vi "Check Registry.vi"(10 "registry":T1[](array[typedef]), 11 "indicator data in":refnum<data-value>) -> (2 "empty registry?":bool, 3 "indicator data out":refnum<data-value>)   [LabVIEW 2018, in "GLog.lvlib" / "UI Updater.lvlib"]
uses:
  UI Updater.lvlib
  Handler Registration.ctl
  Indicator Data.ctl
panel:
  # "Connector Pane"
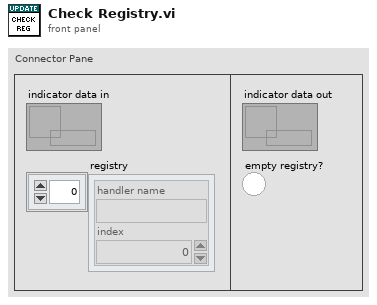
[diagram p1: front panel]
types:
  T1 = typedef "GLog.lvlib/UI Updater.lvlib/Handler Registration.ctl" = cluster{"handler name":string, "index":i32}
  T2 = typedef "GLog.lvlib/UI Updater.lvlib/Indicator Data.ctl" = cluster{"Ctl Ref":refnum<vi>, "Log Buffer":string[], "Log Limit":i32, "Line Limit":i32, "Autoscroll?":bool, "Valid?":bool, "Owning VI":refnum<vi>, "Ctl Index":i32, "Needs Write?":bool}
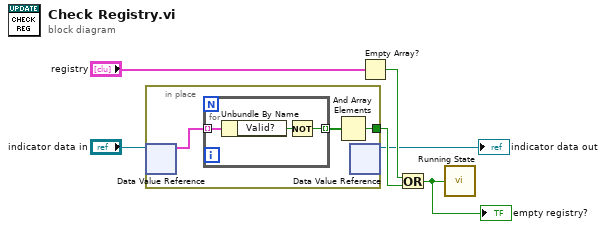
[diagram p0: block diagram]
diagram:
  n1 = in-place {
    in-place-border: [w7] -> w5
    n2 = in-place-dvr #1("indicator data in") -> (w9:T2[])  [unwired: 1 out]
    n3 = for {
      tunnel: w9 -> [w12] mode=indexing
      tunnel: [w10] -> w8 mode=indexing
      n4 = Unbundle By Name(w12) -> ("Valid?"=w11:bool)
      n5 = Not(x=w11) -> (.not. x?=w10:bool)
    }
    n6 = And Array Elements(Boolean array=w8) -> (logical AND=w7:bool)
    n7 = in-place-dvr #1() -> (→"indicator data out":refnum<data-value>)  [unwired: 1 in, 1 out]
  }
  n8 = Empty Array?(array="registry") -> (empty?=w4:bool)
  n9 = Or(x=w4, y=w5) -> (x .or. y?=w6:bool)
  "empty registry?" <- w6
  n10 = call "Running State.vi"("Reset? (F)"=w6) -> ()  [unwired: 1 out]
